vi "SaveCFG.vi"(7 "Clear Before Saving(F)":bool, 8 "error in (no error)":errorcluster, 11 "object in":refnum<class "AIO-Configuration.lvclass">) -> (0 "error out":errorcluster, 2 "OK?":bool, 3 "object out":refnum<class "AIO-Configuration.lvclass">)   [LabVIEW 2021, in "AIO-Channel.lvlib" / "AIO-Configuration.lvclass"]
doc: "Saves Configuration"
uses:
  AIO-Configuration.lvclass
  C:/Users/averna/Documents/LV Gym DEMO/Factory Pattern/Channels/Dependencies/Channel.lvlibp/Channel/Configuration_class/Configuration.lvclass
  Dependencies/Channel.lvlibp/Channel/Configuration_class/properties/ReadConfigurationFile.vi
  <vilib>/Utility/config.llb/Write Key (String).vi
  Dependencies/Channel.lvlibp/Channel/Configuration_class/Configuration.lvclass
  <vilib>/Utility/config.llb/NI_LVConfig.lvlib
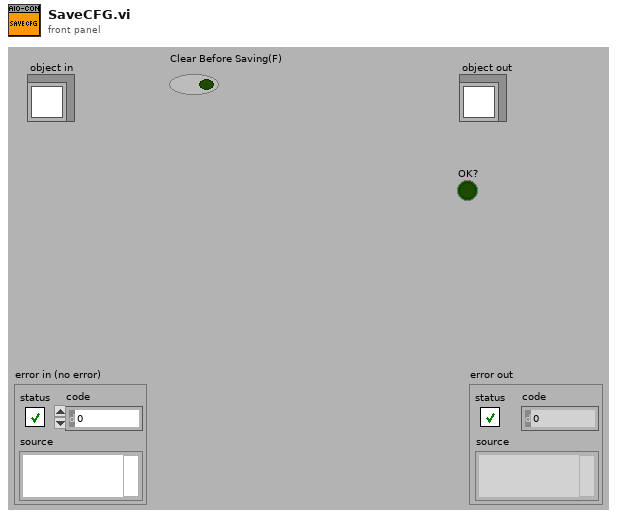
[diagram p1: front panel]
types:
  T1 = typedef "NI_LVConfig.lvlib/Config Data RefNum.ctl" = refnum<k1>
  T2 = typedef "AIO-Channel.lvlib/AIO-Configuration.lvclass/Direction.ctl" = enum16{"Input", "Output"}
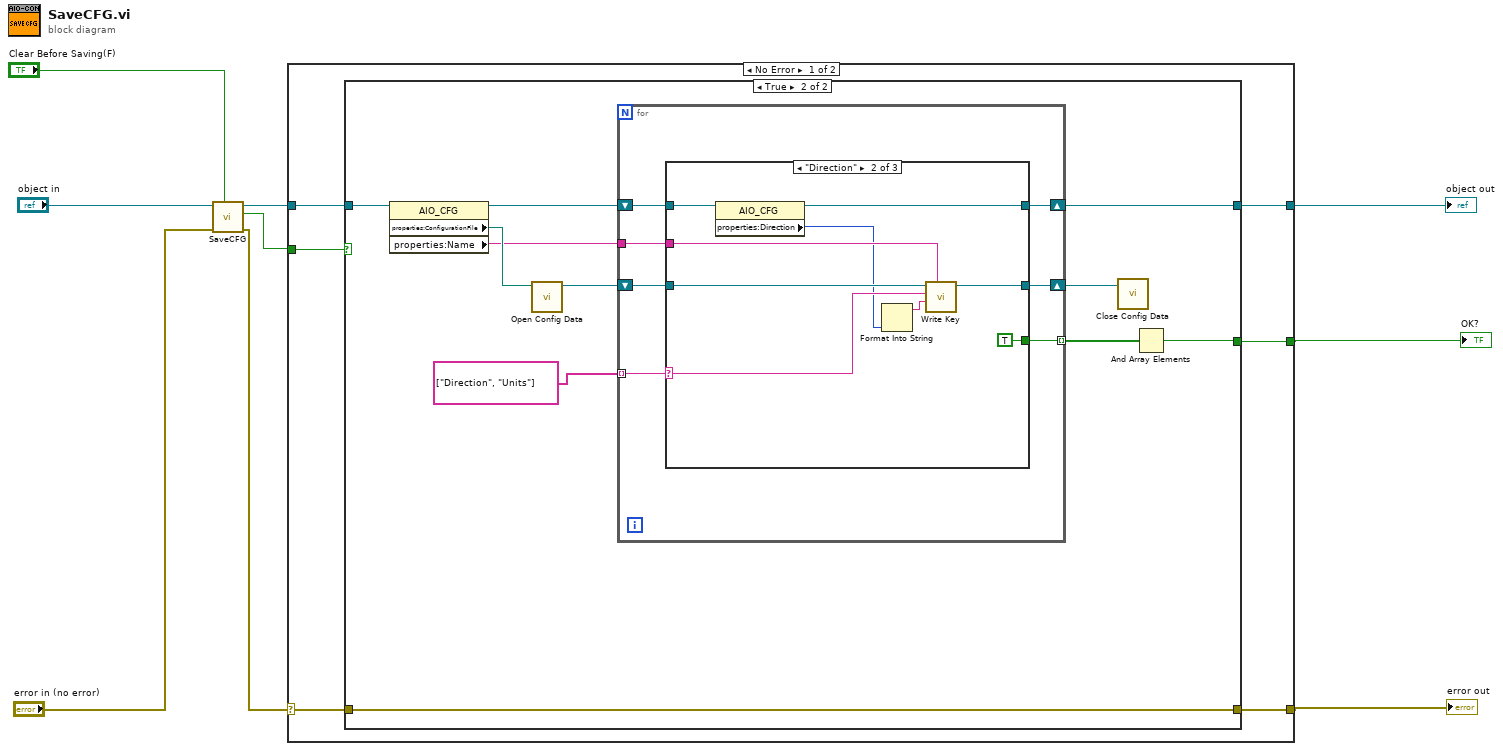
[diagram p0: block diagram]
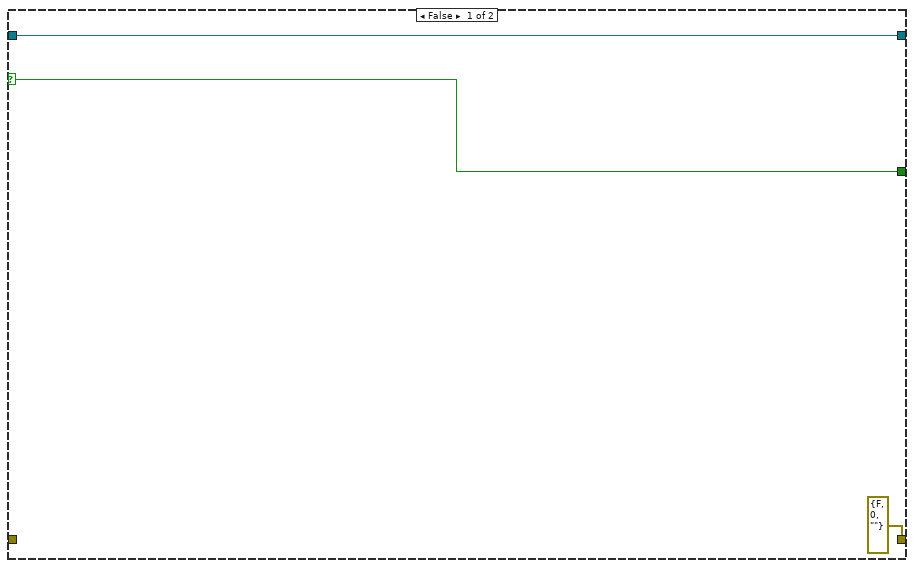
[diagram p2: hidden frame]
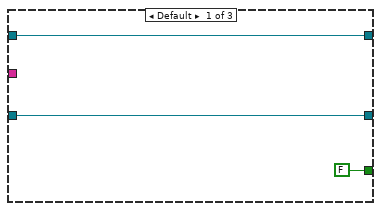
[diagram p3: hidden frame]
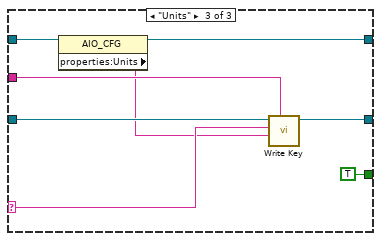
[diagram p4: hidden frame]
diagram:
  n1 = call-parent "SaveCFG.vi"("Clear Before Saving(F)"="Clear Before Saving(F)", "error in (no error)"="error in (no error)", "object in"="object in") -> ("error out"=w1:errorcluster, "OK?"=w2:bool, "object out"=w6:refnum<class "AIO-Configuration.lvclass">)  [unwired: 6 in]
  n2 = case shown="No Error" w1 {
    selector: w1 -> [w12 w59]
    tunnel: [w13 w59] -> w3
    tunnel: w6 -> [w14 w58]
    tunnel: [w10 w57] -> w4
    tunnel: w2 -> [w11 w57]
    tunnel: [w15 w58] -> w5
    frame No Error {
      n3 = case shown="True" w11 {
        selector: w11 -> [w17 _]
        tunnel: [w18 w25] -> w15
        tunnel: w14 -> [w18 w29]
        tunnel: [errorcluster {"status"=FALSE, "code"=0, "source"=""} ("error IO") w28] -> w13
        tunnel: w12 -> [_ w28]
        tunnel: [w17 w19] -> w10
        frame False {
        }
        frame True {
          n4 = property class="AIO_CFG"(reference=w29) -> (reference out=w24:refnum<class "AIO-Configuration.lvclass">, "properties:ConfigurationFile"=w27:path, "properties:Name"=w21:string)  [unwired: 1 in, 1 out]
          n5 = call <vilib>:"Open Config Data.vi"("configuration file path"=w27) -> ("refnum"=w26:T1)  [unwired: 8 in, 2 out]
          n6 = for {
            shift-right: [w32] -> w25
            shift-left: w24 -> [w31]
            shift-right: [w35] -> w23
            shift-left: w26 -> [w36]
            tunnel: string[] ["Direction", "Units"] -> [w34] mode=indexing
            tunnel: w21 -> [w33]
            tunnel: [w30] -> w20 mode=indexing
            n7 = case shown="\"Direction\"" w34 {
              selector: w34 -> [_ w46 w54]
              tunnel: w36 -> [w38 w48 w56]
              tunnel: [w38 w47 w55] -> w35
              tunnel: w33 -> [_ w45 w53]
              tunnel: [w39 w43 w51] -> w32
              tunnel: w31 -> [w39 w44 w52]
              tunnel: [FALSE ("found?") TRUE ("found?") TRUE ("found?")] -> w30
              frame Default {
              }
              frame "Direction" {
                n8 = property class="AIO_CFG"(reference=w44) -> (reference out=w43:refnum<class "AIO-Configuration.lvclass">, "properties:Direction"=w41:T2)  [unwired: 1 in, 1 out]
                n9 = Format Into String(w41) -> (resulting string=w42:string)  [unwired: 3 in, 1 out]
                n10 = call-poly <vilib>:"Write Key.vi"("section"=w45, "value"=w42, "key"=w46, "refnum"=w48) -> ("refnum out"=w47:T1)  [unwired: 5 in, 2 out]
              }
              frame "Units" {
                n11 = property class="AIO_CFG"(reference=w52) -> (reference out=w51:refnum<class "AIO-Configuration.lvclass">, "properties:Units"=w50:string)  [unwired: 1 in, 1 out]
                n12 = call-poly <vilib>:"Write Key.vi"("section"=w53, "value"=w50, "key"=w54, "refnum"=w56) -> ("refnum out"=w55:T1)  [unwired: 5 in, 2 out]
              }
            }
          }
          n13 = call <vilib>:"Close Config Data.vi"("refnum"=w23) -> ()  [unwired: 9 in, 2 out]
          n14 = And Array Elements(Boolean array=w20) -> (logical AND=w19:bool)
        }
      }
    }
    frame Error {
    }
  }
  "error out" <- w3
  "object out" <- w5
  "OK?" <- w4
